vi "Do.vi"(8 "error in (no error)":errorcluster, 10 "Actor in":refnum<class "Actor.lvclass">, 11 "Store Measuement Config Msg":refnum<class "Store Measuement Config Msg.lvclass">) -> (0 "error out":errorcluster, 2 "Actor out":refnum<class "Actor.lvclass">)   [LabVIEW 2017, in "Measurement Setup Controller.lvlib" / "Store Measuement Config Msg.lvclass"]
doc: "This VI delivers the message to the actor by calling the appropriate method(s) on the actor."
uses:
  Store Measuement Config Msg.lvclass
  <vilib>/ActorFramework/Actor/Actor.lvclass
  Measurement Setup.lvclass
  C:/Program Files (x86)/National Instruments/LabVIEW 2017/vi.lib/ActorFramework/Actor/Actor.lvclass
  C:/Program Files (x86)/National Instruments/LabVIEW 2017/user.lib/Common Components/Controller/Controller.lvclass
  Store Measuement Config Msg.lvclass/Store Measuement Config Msg.ctl
  Measurement Data/Measurement Data.lvclass/Measurement Data.ctl
  <userlib>/Common Components/Measurement Actor/Measurement.lvclass/Measurement.ctl
  Measurement Setup.lvclass/Measurement Setup.ctl
  <vilib>/ActorFramework/Actor/Actor.lvclass/Actor.ctl
  <vilib>/ActorFramework/Message Enqueuer/Message Enqueuer.lvclass/Message Enqueuer.ctl
  <vilib>/ActorFramework/Actor/Read Self Enqueuer.vi
  <vilib>/ActorFramework/Stop Msg/Send Normal Stop.vi
  Measurement Data/Write Step Configuration.vi
  Measurement Data/Read Device Names.vi
  <userlib>/Common Components/Measurement Actor/Accessors/Read Step Configuration.vi
  Measurement Data/Write Array of Device Configuration.vi
  Measurement Data/Read Measurement Name.vi
  <vilib>/ActorFramework/Message Enqueuer/Init from Existing Queue.vi
  <vilib>/ActorFramework/Message Enqueuer/Enqueue.vi
  <vilib>/ActorFramework/Stop Msg/Stop Msg.lvclass
  C:/Program Files (x86)/National Instruments/LabVIEW 2017/vi.lib/ActorFramework/Message/Message.lvclass
  <userlib>/Common Components/Controller/Methods/Lookup Hardware by Name.vi
  <userlib>/Common Components/Controller/Methods/Lookup Measurement by Name.vi
  <vilib>/ActorFramework/Message Priority Queue/Priority Enqueue.vi
  <userlib>/Common Components/Measurement Actor/Configuration/Step Configuration.lvclass
  <vilib>/ActorFramework/Message Enqueuer/Message Enqueuer.lvclass
  <userlib>/Common Components/Hardware/Hardware.lvclass
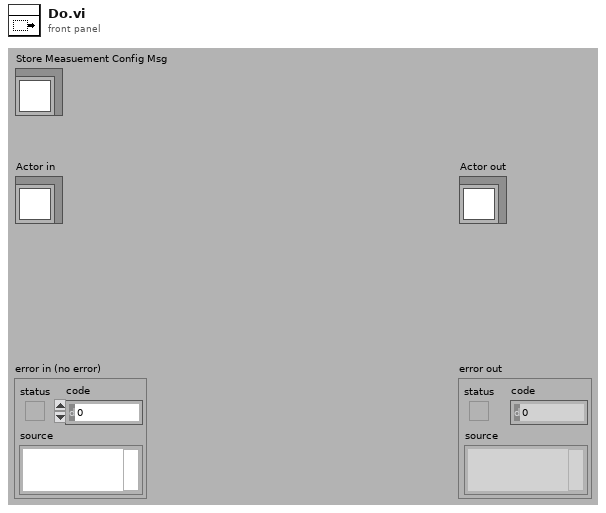
[diagram p1: front panel]
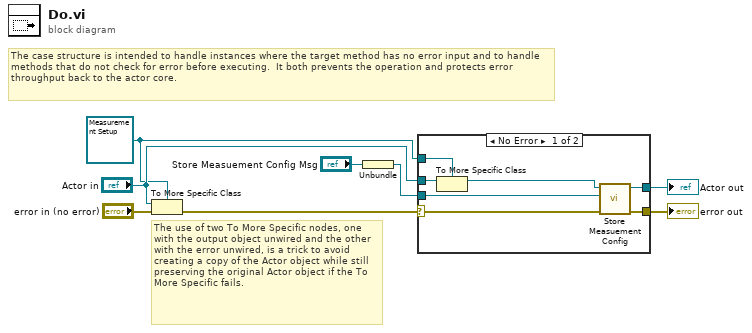
[diagram p0: block diagram]
diagram:
  w2 = refnum<class "Measurement Setup.lvclass"> refnum ("Actor in")
  # "The use of two To More Specific nodes, one with the output object unwired and the other with the error unwired, is a trick to avoid creating a copy of the Actor object while still preserving the original Actor object if the To More Specific fails."
  # "The case structure is intended to handle instances where the target method has no error input and to handle methods that do not check for error before executing.  It both prevents the operation and protects error throughput back to the actor core."
  n1 = To More Specific Class(target class=w2, reference="Actor in", error in="error in (no error)") -> (error out=w6:errorcluster)  [unwired: 1 out]
  n2 = Unbundle("Store Measuement Config Msg") -> (w1:refnum<class "Measurement Data.lvclass">)
  n3 = case shown="No Error" w6 {
    selector: w6 -> [w13 w17]
    tunnel: [w15 w17] -> w5
    tunnel: [w14 w16] -> w4
    tunnel: "Actor in" -> [w12 w16]
    tunnel: w2 -> [w11 _]
    tunnel: w1 -> [w9 _]
    frame No Error {
      n4 = To More Specific Class(target class=w11, reference=w12) -> (specific class reference=w10:refnum<class "Measurement Setup.lvclass">)  [unwired: 1 in, 1 out]
      n5 = call "Store Measuement Config.vi"("error in (no error)"=w13, "Measurement Setup Controller.lvlib:Measurement Data.lvclass"=w9, "Measurement Setup in"=w10) -> ("error out"=w15:errorcluster, "Measurement Setup out"=w14:refnum<class "Measurement Setup.lvclass">)  [unwired: 7 in]
    }
    frame Error {
      # "If type check fails, pass the original object out again."
    }
  }
  "error out" <- w5
  "Actor out" <- w4
